vi "VIH Project Tree - Delete Items.vi"(8 "error in":errorcluster, 10 "Tree Item Tags":string[](array[string]), 11 "Project Tree":T1) -> (0 "error out":errorcluster, 3 "dup Project Tree":T1)   [LabVIEW 2014]
doc: "::: VI Helpeks :::\nCopyright (c) 2000-2026 Konstantin Shifershteyn. All rights reserved."
uses:
  VIH Project Tree Typedef - Tree Refnum.ctl
panel:
  # "VI Helpeks\nCopyright (c) 2012-2026 Konstantin Shifershteyn"
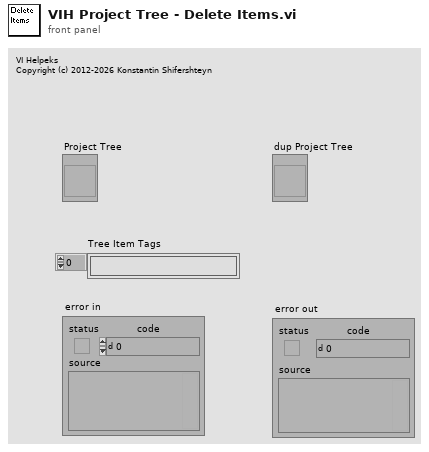
[diagram p1: front panel]
types:
  T1 = typedef "VIH Project Tree Typedef - Tree Refnum.ctl" = refnum<vi>
  T2 = typedef "VIH HelpGen Typedef - Palette - Item Type Enum.ctl" = enum32{"<Invalid>", "<unknown>", "VI", "Menu", "LV Func", "Express VI", "Poly VI", "CTL", "HTML"}
  T3 = cluster{"Types":T2[], "Paths":path[], "Dynamic":enum16{"Dyn", "Stat", "Both"}[], "Can be built":bool[], "DynFileNotFound":bool[]}
  T4 = enum16{"get", "get all", "set", "Init", "delete"}
  T5 = enum16{"get", "get all", "set", "Init", "delete", "rename"}
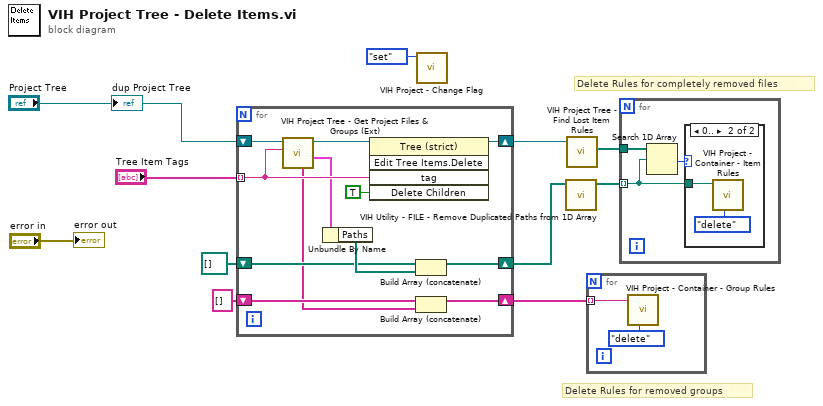
[diagram p0: block diagram]
diagram:
  # "Delete Rules for completely removed files"
  # "Delete Rules for removed groups"
  n1 = for {
    tunnel: "Tree Item Tags" -> [w19] mode=indexing
    shift-right: [w22] -> w5
    shift-left: "Project Tree" -> [w21]
    shift-right: [w15] -> w10
    shift-left: path[] [] -> [w16]
    shift-right: [w12] -> w9
    shift-left: string[] [] -> [w14]
    n2 = call "VIH Project Tree - Get Project Files & Groups (Ext).vi"("Parent Item Tag (Root)"=w19, "Project Tree"=w21) -> ("Project Files"=w18:T3, "dup Project Tree"=w20:T1, "Project Group IDs"=w13:string[])  [unwired: 6 in, 1 out]
    n3 = Unbundle By Name(w18) -> ("Paths"=w17:path[])
    n4 = invoke class="Tree (strict)" method="Edit Tree Items.Delete"(reference=w20, "tag"=w19, "Delete Children"=TRUE) -> (reference out=w22:T1)  [unwired: 2 in, 4 out]
    n5 = Build Array (concatenate)(w16, w17) -> (w15:path[])
    n6 = Build Array (concatenate)(w14, w13) -> (w12:string[])
  }
  n7 = call "VIH Project - Change Flag.vi"("cmd (get)"=enum16{"get", "set", "reset"}."set") -> ()  [unwired: 9 in, 2 out]
  n8 = call "VIH Utility - FILE - Remove Duplicated Paths from 1D Array.vi"("Array in"=w10) -> ("Array out"=w11:path[])  [unwired: 9 in, 1 out]
  n9 = call "VIH Project Tree - Find Lost Item Rules.vi"("Project Tree"=w5) -> ("Lost Rules (Owner Paths)"=w7:path[])  [unwired: 8 in, 2 out]
  n10 = for {
    tunnel: w9 -> [w25] mode=indexing
    n11 = call "VIH Project - Container - Group Rules.vi"("cmd (get)"=T4."delete", "Group ID"=w25) -> ()  [unwired: 5 in, 5 out]
  }
  n12 = for {
    tunnel: w11 -> [w28] mode=indexing
    tunnel: w7 -> [w27]
    n13 = Search 1D Array(1D array=w27, element=w28) -> (index of element=w26:i32)  [unwired: 1 in]
    n14 = case shown="0.." w26 {
      tunnel: w28 -> [_ w29]
      frame ..-1 {
      }
      frame 0.. {
        n15 = call "VIH Project - Container - Item Rules.vi"("cmd (get)"=T5."delete", "Item Path"=w29) -> ()  [unwired: 5 in, 5 out]
      }
    }
  }
  "dup Project Tree" <- "Project Tree"
  "error out" <- "error in"
